vi "UN_folder_ex.vi"(8 "error in":errorcluster, 11 "path":path) -> (0 "error out":errorcluster, 1 "Array":path[](array[path]), 2 "logical OR":bool, 3 "foldername":string[](array[string]))   [LabVIEW 2018]
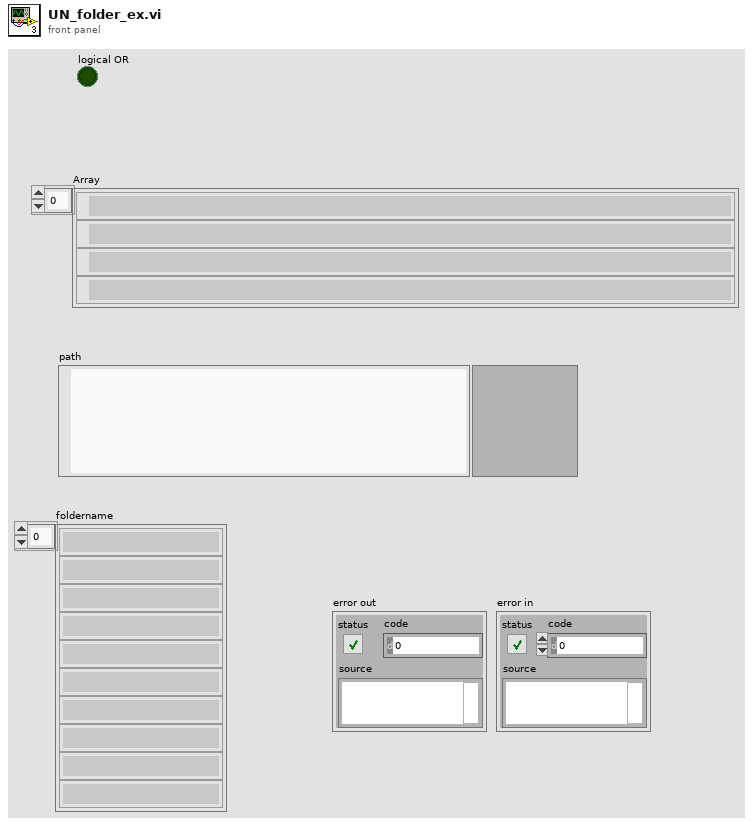
[diagram p1: front panel]
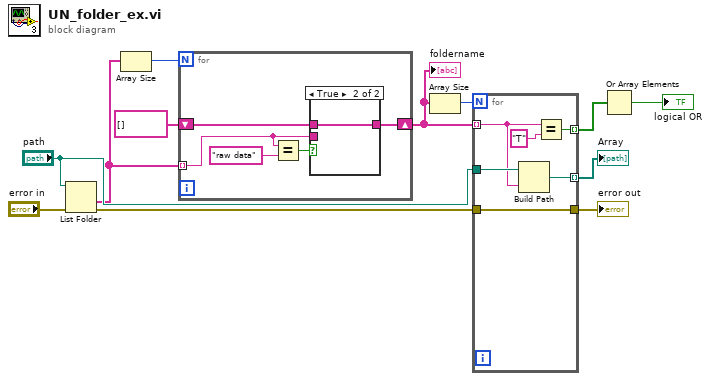
[diagram p0: block diagram]
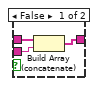
[diagram p2: hidden frame]
diagram:
  n1 = List Folder(path="path", error in="error in") -> (folder names=w4:string[], error out=w10:errorcluster)  [unwired: 2 in, 2 out]
  n2 = Array Size(array=w4) -> (size(s)=w6:i32)
  n3 = for {
    N: w6 -> [_]
    tunnel: w4 -> [w15] mode=indexing
    shift-right: [w14] -> w3
    shift-left: string[] [] -> [w13]
    n4 = Equal?(x=w15, y="raw data") -> (x = y?=w16:bool)
    n5 = case shown="True" w16 {
      tunnel: w15 -> [w20 _]
      tunnel: [w19 w21] -> w14
      tunnel: w13 -> [w18 w21]
      frame False {
        n6 = Build Array (concatenate)(w18, w20) -> (w19:string[])
      }
      frame True {
      }
    }
  }
  "foldername" <- w3
  n7 = Array Size(array=w3) -> (size(s)=w11:i32)
  n8 = for {
    N: w11 -> [_]
    tunnel: w3 -> [w23] mode=indexing
    tunnel: w10 -> [w25]
    tunnel: [w26] -> w9 mode=indexing
    tunnel: [w25] -> w1
    tunnel: "path" -> [w24]
    tunnel: [w22] -> w7 mode=indexing
    n9 = Build Path(base path=w24, name or relative path=w23) -> (appended path=w22:path)
    n10 = Equal?(x=w23, y="T" ("regular expression")) -> (x = y?=w26:bool)
  }
  "error out" <- w1
  "Array" <- w7
  n11 = Or Array Elements(Boolean array=w9) -> (logical OR=→"logical OR":bool)
